vi "Initialization.vi"(8 "error in":errorcluster, 9 "UI Refs":T1, 10 "user event":T2, 11 "Hydraulic in":refnum<class "H1 Hydraulic.lvclass">) -> (0 "error out":errorcluster, 3 "Hydraulic out":refnum<class "H1 Hydraulic.lvclass">)   [LabVIEW 2025, in "H1 Plotter.lvlib" / "H1 Hydraulic.lvclass"]
uses:
  H1 Hydraulic.lvclass
  Users/Public/Documents/Sandia National Labs/TSS Plugin/CEF.lvlibp/Node/UserEventRef.ctl
  H1 Hydraulic.lvclass/H1 Hydraulic.ctl
  Users/Public/Documents/Sandia National Labs/TSS Plugin/Tests/XY Plotter.lvlibp/XY  Plotter/XY Plotter.lvclass
  Users/Public/Documents/Sandia National Labs/TSS Plugin/CEF.lvlibp/Node/CEF_Node.lvclass
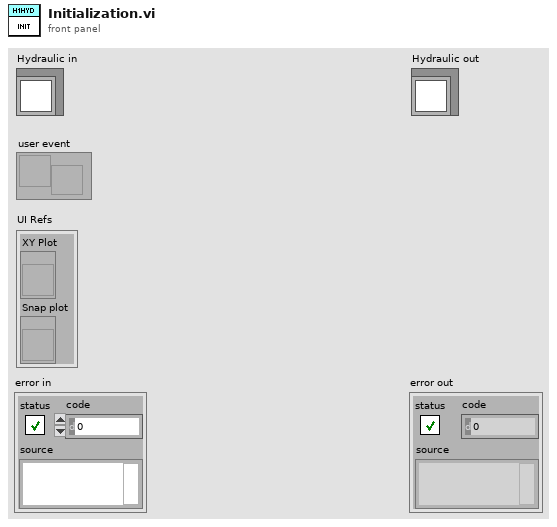
[diagram p1: front panel]
types:
  T1 = cluster{"XY Plot":refnum<vi>, "Snap plot":refnum<vi>}
  T2 = typedef "CEF.lvlibp/CEF_Node.lvclass/UserEventRef.ctl" = refnum<user-event>
  T3 = cluster{"Name":string, "Color":u32, "Style":u8, "Point Style":u8, "Name Visible":bool, "Allow Drag":bool, "Annotation Mode":u32, "Plot":i32, "Index":i32, "Position":cluster{"X":dbl, "Y":dbl}, "X Scale":u32, "Y Scale":u32, "Show Arrow":bool, "Lock Name":bool, "Plot Area":i32, "Label Offset":cluster{"X":dbl, "Y":dbl}}
  T4 = cluster{"Name":string, "Color":u32, "Style":u8, "Point Style":u8, "Name Visible":bool, "Allow Drag":bool, "Annotation Mode":u32, "Plot":i32, "Index":i32, "Position":cluster{"X":dbl, "Y":dbl}, "X Scale":u32, "Y Scale":u32, "Show Arrow":bool, "Lock Name":bool, "Plot Area":i32, "Label Offset":cluster{"X":dbl, "Y":dbl}}[]
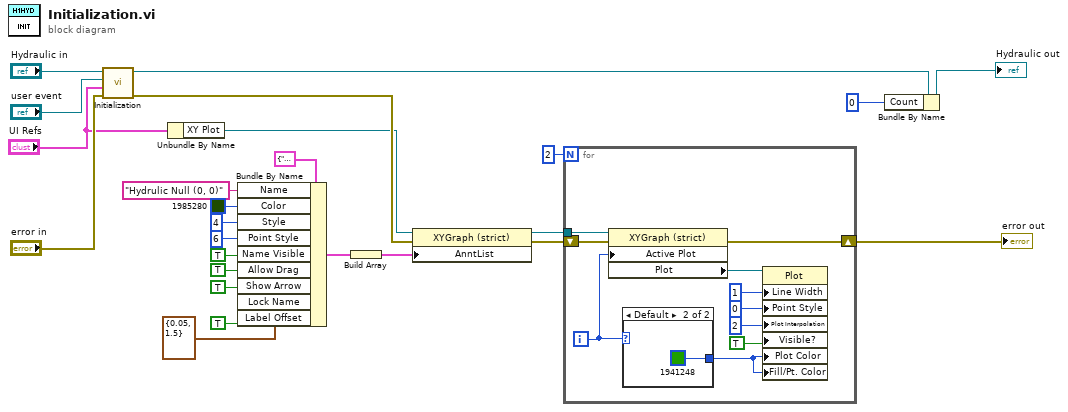
[diagram p0: block diagram]
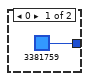
[diagram p2: hidden frame]
diagram:
  n1 = call-parent "Initialization.vi"("error in"="error in", "UI Refs"="UI Refs", "user event"="user event", "XY Plotter"="Hydraulic in") -> ("error out"=w8:errorcluster, "XY Plotter out"=w25:refnum<class "H1 Hydraulic.lvclass">)  [unwired: 6 in]
  n2 = Unbundle By Name("UI Refs") -> ("XY Plot"=w5:refnum<vi>)
  n3 = Bundle By Name(cluster=T3 {"Name"="", "Color"=0, "Style"=0, "Point Style"=0, "Name Visible"=FALSE, "Allow Drag"=FALSE, "Annotation Mode"=0, "Plot"=0, "Index"=0, "Position"={"X"=0.0, "Y"=0.0}, "X Scale"=0, "Y Scale"=0, "Show Arrow"=FALSE, "Lock Name"=FALSE, "Plot Area"=0, "Label Offset"={"X"=0.0, "Y"=0.0}}, "Name"="Hydrulic Null (0, 0)" ("Hydraulic Null"), "Color"=u32 1985280, "Style"=u8 4, "Point Style"=u8 6, "Name Visible"=TRUE, "Allow Drag"=TRUE, "Show Arrow"=TRUE, "Lock Name"=TRUE, "Label Offset"=cluster{"X":dbl, "Y":dbl} {"X"=0.05, "Y"=1.5}) -> (w12:T3)
  n4 = Build Array(w12) -> (w10:T4)
  n5 = property class="XYGraph (strict)"(reference=w5, error in=w8, "AnntList"=w10) -> (reference out=w1:refnum<vi>, error out=w4:errorcluster)
  n6 = for {
    N: 2 -> [_]
    tunnel: w1 -> [w35]
    shift-right: [w26] -> w2
    shift-left: w4 -> [w30]
    i -> [w28]
    n7 = property class="XYGraph (strict)"(reference=w35, error in=w30, "Active Plot"=w28) -> (error out=w26:errorcluster, "Plot"=w31:refnum<vi>)  [unwired: 1 out]
    n8 = case shown="Default" w28 {
      tunnel: [u32 3381759 ("Plot Color") u32 1941248 ("Plot Color")] -> w27
      frame 0 {
      }
      frame Default {
      }
    }
    n9 = property class="Plot"(reference=w31, "Line Width"=u8 1, "Point Style"=u8 0, "Plot Interpolation"=u8 2, "Visible?"=TRUE ("Visible"), "Plot Color"=w27, "Fill/Pt. Color"=w27) -> ()  [unwired: 1 in, 2 out]
  }
  "error out" <- w2
  n10 = Bundle By Name(cluster=w25, "Count"=0) -> (→"Hydraulic out":refnum<class "H1 Hydraulic.lvclass">)
